vi "RFH-utility-compare_double.vi"(7 "% tolerance (0.1)":dbl=0.1, 10 "New":dbl, 11 "original":dbl) -> (2 "In Range?":bool)   [LabVIEW 2020, in "RFH-Reflection_File_Handler.lvlib"]
doc: "Checks whether a new value lies within a percent tolerance (default 0.1) of the original value."
uses:
  RFH-Reflection_File_Handler.lvlib
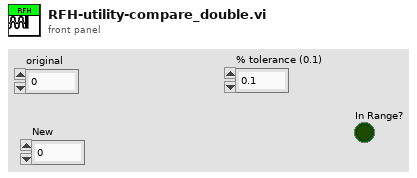
[diagram p1: front panel]
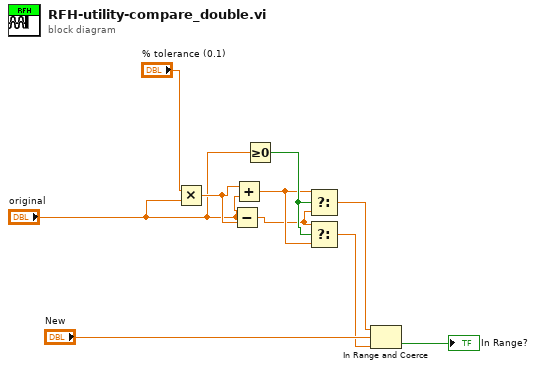
[diagram p0: block diagram]
diagram:
  n1 = Multiply(x="% tolerance (0.1)", y="original") -> (x*y=w9:dbl)
  n2 = Subtract(x="original", y=w9) -> (x-y=w3:dbl)
  n3 = Add(x=w9, y="original") -> (x+y=w4:dbl)
  n4 = Greater Or Equal To 0?(x="original") -> (x >= 0?=w5:bool)
  n5 = Select(t=w4, s=w5, f=w3) -> (s? t:f=w2:dbl)
  n6 = Select(t=w3, s=w5, f=w4) -> (s? t:f=w1:dbl)
  n7 = In Range and Coerce(upper limit=w2, x="New", lower limit=w1) -> (In Range?=→"In Range?":bool)  [unwired: 1 out]
